vi "Run Runnable.vi"(8 "error in (no error)":errorcluster, 10 "Runnable":refnum<class "Runnable.lvclass">, 11 "Single Thread Test Runner In":refnum<class "Single Thread Test Runner.lvclass">) -> (0 "error out":errorcluster, 3 "Single Thread Test Runner Out":refnum<class "Single Thread Test Runner.lvclass">)   [LabVIEW 2020, in "Single Thread Test Runner.lvclass"]
uses:
  Single Thread Test Runner.lvclass
  Execute.vi
  Runnable.lvclass
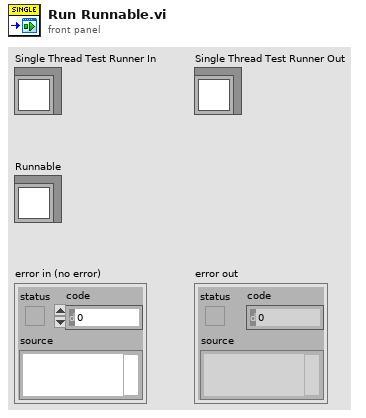
[diagram p1: front panel]
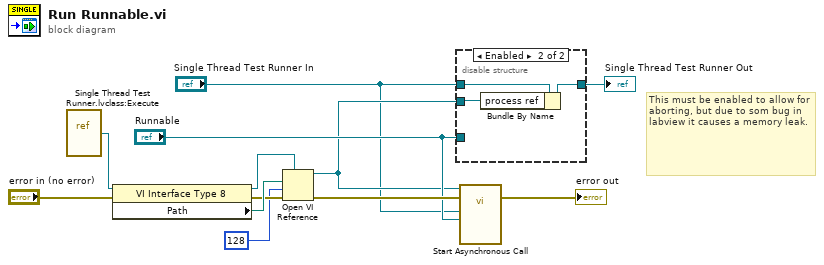
[diagram p0: block diagram]
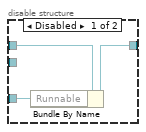
[diagram p2: hidden frame]
diagram:
  # "This must be enabled to allow for aborting, but due to som bug in labview it causes a memory leak."
  n1 = vi-ref "Single Thread Test Runner.lvclass:Execute.vi"() -> (w12:refnum<vi>)
  n2 = property class="VI Interface Type 8"(reference=w12, error in="error in (no error)") -> (reference out=w10:refnum<vi>, error out=w9:errorcluster, "Path"=w11:path)
  n3 = Open VI Reference(type specifier VI Refnum (for type only)=w10, vi path=w11, options=128, error in (no error)=w9) -> (vi reference=w2:refnum<vi>, error out=w7:errorcluster)  [unwired: 2 in]
  n4 = disable-structure shown="Enabled" {
    disable-tunnel: "Single Thread Test Runner In" -> [w15 w18]
    disable-tunnel: [w14 w17] -> w4
    disable-tunnel: "Runnable" -> [w13 _]
    disable-tunnel: w2 -> [_ w16]
    frame Disabled {
      n5 = Bundle By Name(cluster=w15, "Runnable"=w13) -> (w14:refnum<class "Single Thread Test Runner.lvclass">)
    }
    frame Enabled {
      n6 = Bundle By Name(cluster=w18, "process ref"=w16) -> (w17:refnum<class "Single Thread Test Runner.lvclass">)
    }
  }
  "Single Thread Test Runner Out" <- w4
  n7 = call-by-ref "Start Asynchronous Call"(reference=w2, error in=w7, "Test Runner V2 in"="Runnable", "Single Thread Test Runner.lvclass"="Single Thread Test Runner In") -> (error out=→"error out":errorcluster)  [unwired: 10 in, 1 out]
